vi "Configure ECAT Generic Slave.vi"(8 "error in":errorcluster, 10 "Distributed Clock":bool, 11 "IOV ref":refnum<k21>) -> (0 "error out":errorcluster, 2 "Distributed Clock out":bool, 3 "IOV ref out":refnum<k21>)   [LabVIEW 2027, in "SEECD Engine.lvlib"]
uses:
  SEECD Engine.lvlib
  <resource>/objmgr/IndComECAT.rc
  <vilib>/NI VeriStand/Custom Device Tools/Custom Device Utility Library/Custom Device Utility Library.lvlib
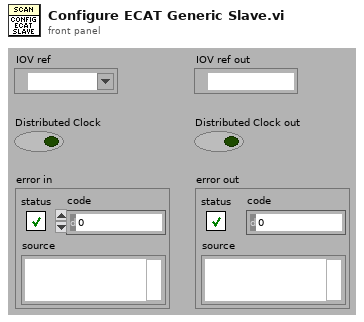
[diagram p1: front panel]
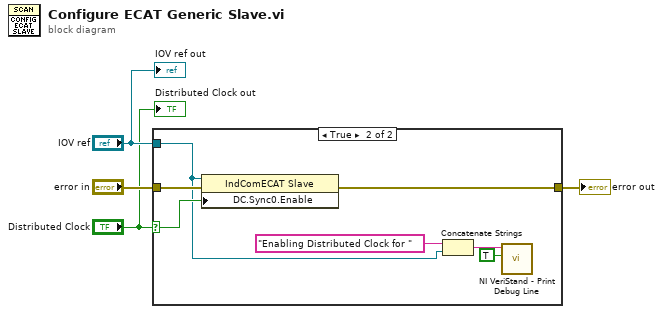
[diagram p0: block diagram]
diagram:
  n1 = case shown="True" "Distributed Clock" {
    selector: "Distributed Clock" -> [_ w10]
    tunnel: [w5 w12] -> w4
    tunnel: "error in" -> [w5 w11]
    tunnel: "IOV ref" -> [_ w9]
    frame False {
    }
    frame True {
      n2 = property class="IndComECAT Slave"(reference=w9, error in=w11, "DC.Sync0.Enable"=w10) -> (error out=w12:errorcluster)  [unwired: 1 out]
      n3 = Concatenate Strings("Enabling Distributed Clock for ", w9) -> (w7:string)
      n4 = call <vilib>:"NI VeriStand - Print Debug Line.vi"("Add to log file? (F)"=TRUE, "Message"=w7) -> ()  [unwired: 9 in, 1 out]
    }
  }
  "error out" <- w4
  "IOV ref out" <- "IOV ref"
  "Distributed Clock out" <- "Distributed Clock"
